vi "Search.vi"() -> (8 "data":string[][](array[string]), 10 "Leds":bool[](array[boolean]))   [LabVIEW 2021]
uses:
  <vilib>/addons/_office/excel.llb/Excel Get Data ([str]).vi
  <vilib>/Utility/NIReport.llb/NI_report.lvclass
  <vilib>/Utility/NIReport.llb/Excel/NI_Excel.lvclass
  <vilib>/addons/_office/NI_ReportGenerationToolkit.lvlib
panel:
  in  "Check":bool
  in  "Saisir des chiffres\nvérifier":string[](array[string])
  out "data string":string[][](array[string])
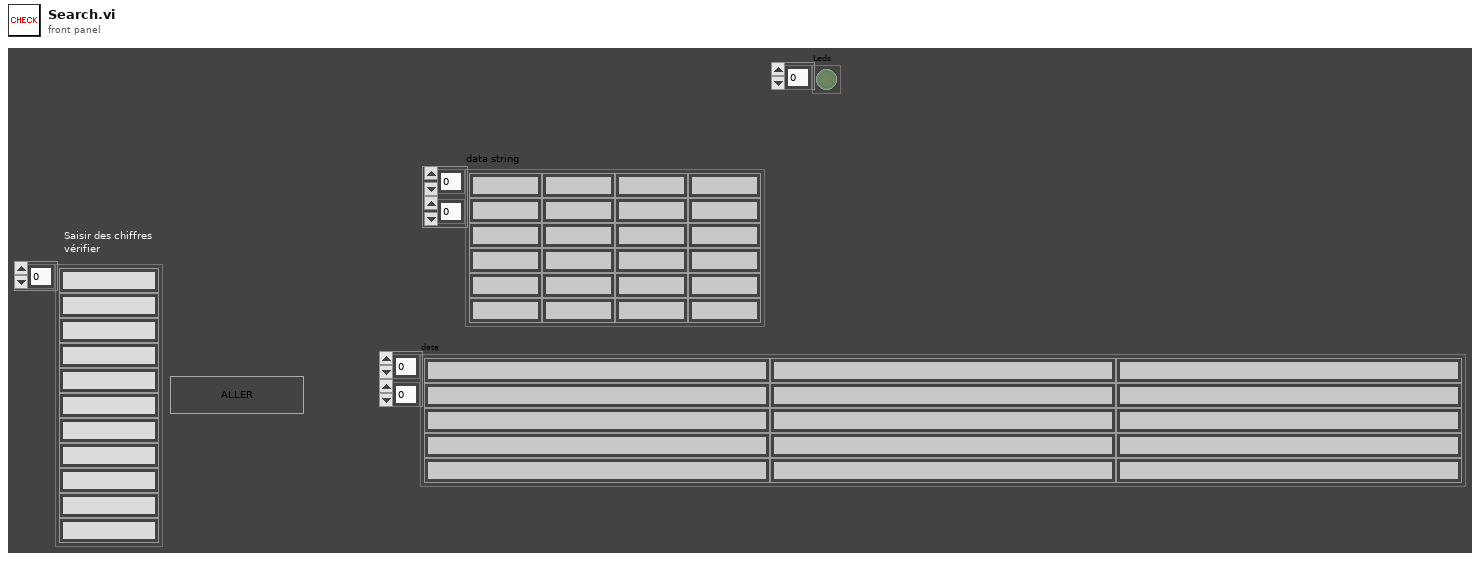
[diagram p1: front panel]
types:
  T1 = enum16{"Standard Report", "HTML", "Word", "Excel"}
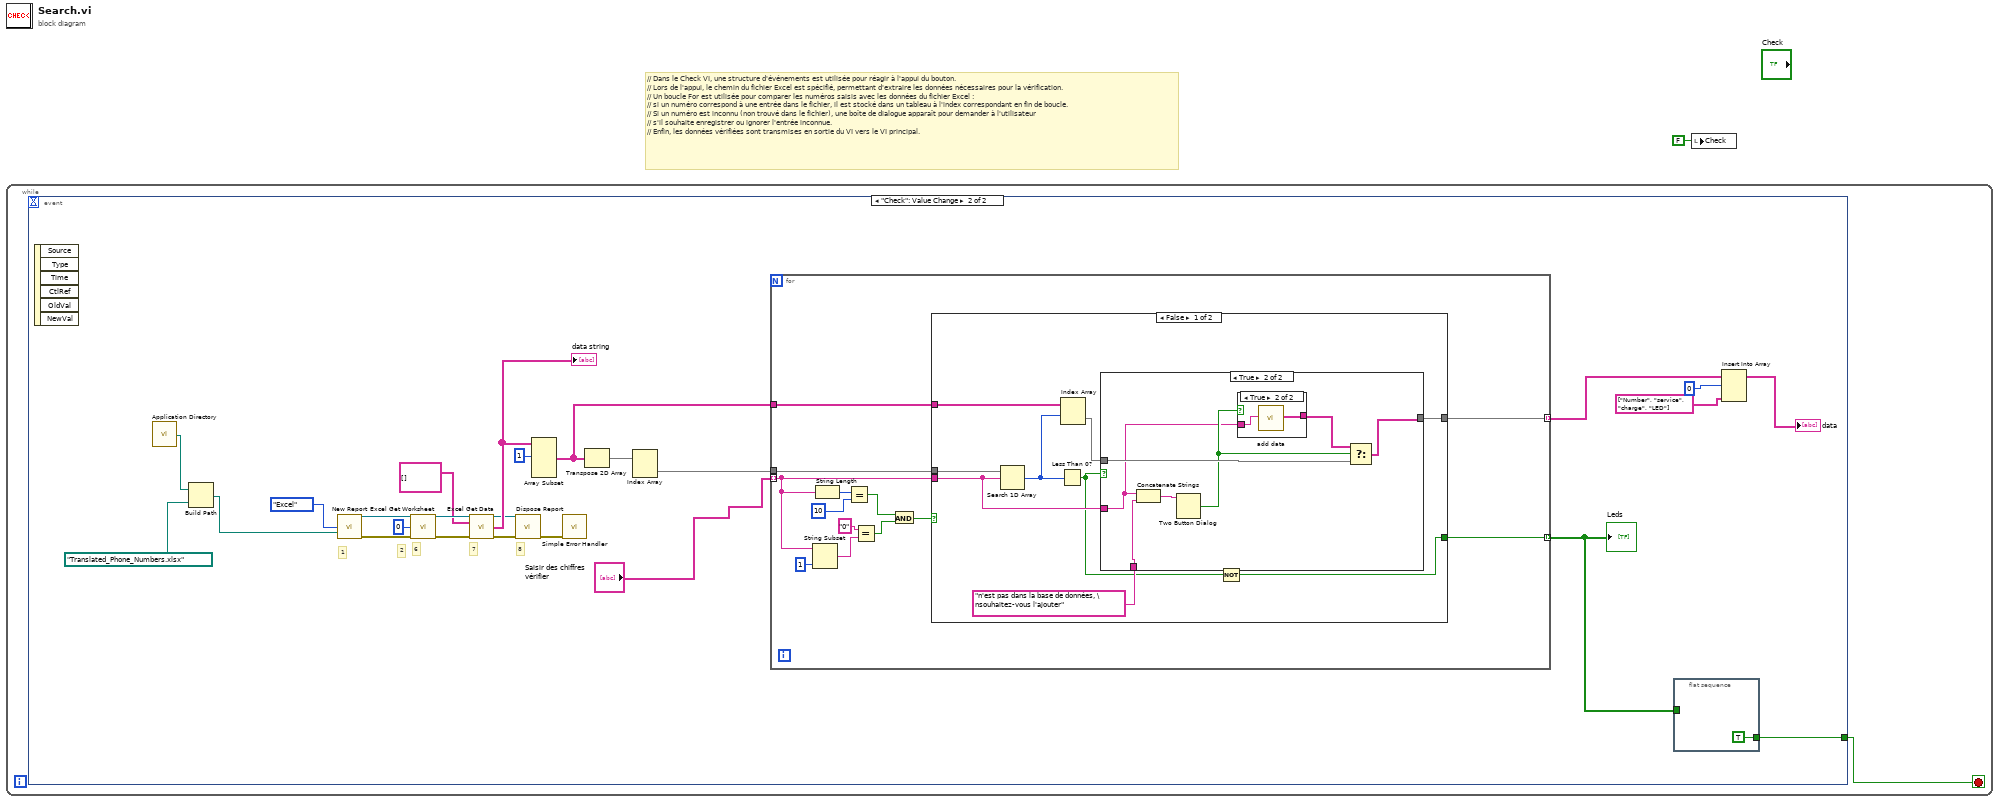
[diagram p0: block diagram]
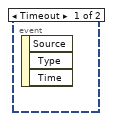
[diagram p2: hidden frame]
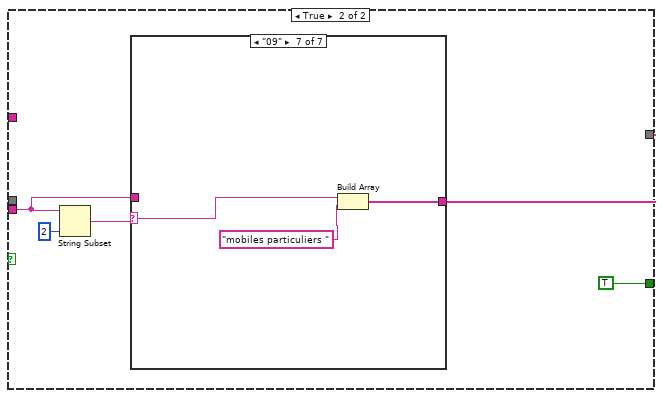
[diagram p5: hidden frame]
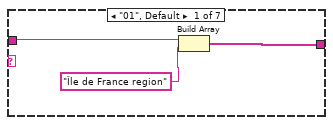
[diagram p6: hidden frame]
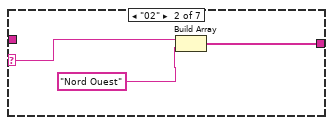
[diagram p7: hidden frame]
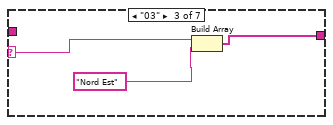
[diagram p8: hidden frame]
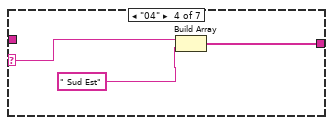
[diagram p9: hidden frame]
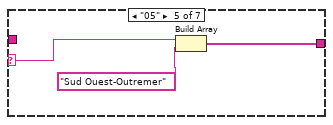
[diagram p10: hidden frame]
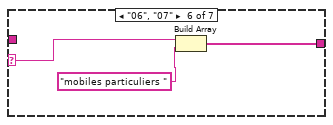
[diagram p11: hidden frame]
diagram:
  # "// Dans le Check VI, une structure d'événements est utilisée pour réagir à l'appui du bouton.\n// Lors de l'appui, le chemin du fichier Excel est spécifié, permettant d'extraire les données nécessaires pour la vérification.\n// Un boucle For est utilisée pour comparer les numéros saisis avec les données du fichier Excel : \n// si un numéro correspond à une entrée dans le fichier, il est stocké dans un tableau à l'index correspondant en fin de boucle.\n// Si un numéro est inconnu (non trouvé dans le fichier), une boîte de dialogue apparaît pour demander à l'utilisateur \n// s'il souhaite enregistrer ou ignorer l'entrée inconnue.\n// Enfin, les données vérifiées sont transmises en sortie du VI vers le VI principal."
  n1 = while {
    stop <- w2 stop-if-true
    n2 = event shown="[1] \"Check\": Value Change" {
      selector: _ -> [_ _]
      dyn-events: _ -> [_ _]
      timeout: _ -> [_ _]
      tunnel: [_ w7] -> w2
      event Timeout {
        n3 = event-data() -> ()  [unwired: 1 in, 3 out]
      }
      event "Check": Value Change {
        # "8"
        # "7"
        # "6"
        # "2"
        # "1"
        n4 = event-data() -> ()  [unwired: 1 in, 6 out]
        n5 = call <vilib>:"Application Directory.vi"() -> ("Application Directory"=w5:path)
        n6 = Build Path(base path=w5, name or relative path=path "Translated_Phone_Numbers.xlsx") -> (appended path=w3:path)
        n7 = call <vilib>:"New Report.vi"("report type"=T1."Excel", "template (empty)"=w3) -> ("report out"=w19:refnum<class "NI_report.lvclass">, "error out"=w20:errorcluster)  [unwired: 12 in]
        n8 = call <vilib>:"Excel Get Worksheet.vi"("report in"=w19, "worksheet index (0)"=0, "error in (no error)"=w20) -> ("report out"=w15:refnum<class "NI_report.lvclass">, "error out"=w14:errorcluster)  [unwired: 11 in]
        n9 = call-poly <vilib>:"Excel Get Data.vi"("report in"=w15, "data type"=string[][] [], "error in (no error)"=w14) -> ("report out"=w16:refnum<class "NI_report.lvclass">, "data"=w23:string[][], "error out"=w17:errorcluster)  [unwired: 10 in]
        "data string" <- w23
        n10 = call-dynamic "Dispose Report.vi"("report in"=w16, "error in (no error)"=w17) -> ("error out"=w18:errorcluster)  [unwired: 13 in]
        n11 = Array Subset(array=w23, index (row)=1 ("index")) -> (w24:string[][])  [unwired: 3 in]
        n12 = call <vilib>:"Simple Error Handler.vi"("error in (no error)"=w18) -> ()  [unwired: 4 in, 5 out]
        n13 = Transpose 2D Array(2D array=w24) -> (transposed array=w21:string[][])
        n14 = Index Array(array=w21) -> (element=w22:string[])  [unwired: 2 in]
        n15 = for {
          tunnel: w22 -> [w41]
          tunnel: "Saisir des chiffres\nvérifier" -> [w34] mode=indexing
          tunnel: w24 -> [w40]
          tunnel: [w39] -> w25 mode=indexing
          tunnel: [w29] -> w6 mode=indexing
          n16 = String Subset(string=w34, length (rest)=1 ("length (rest)")) -> (substring=w37:string)  [unwired: 1 in]
          n17 = String Length(string=w34) -> (length=w33:i32)
          n18 = Equal?(x=w33, y=10) -> (x = y?=w31:bool)
          n19 = Equal?(x="0", y=w37) -> (x = y?=w35:bool)
          n20 = And(x=w31, y=w35) -> (x .and. y?=w30:bool)
          n21 = case shown="False" w30 {
            tunnel: w41 -> [w50 _]
            tunnel: w34 -> [w47 w62]
            tunnel: w40 -> [w49 _]
            tunnel: [w44 w63] -> w39
            tunnel: [w42 TRUE] -> w29
            frame False {
              n22 = Search 1D Array(1D array=w50, element=w47) -> (index of element=w48:i32)  [unwired: 1 in]
              n23 = Less Than 0?(x=w48) -> (x < 0?=w43:bool)
              n24 = Index Array(array=w49, index (row)=w48) -> (element=w45:string[])  [unwired: 1 in]
              n25 = case shown="True" w43 {
                tunnel: w47 -> [_ w52]
                tunnel: "n'est pas dans la base de données, \nsouhaitez-vous l'ajouter" ("string") -> [_ w58]
                tunnel: w45 -> [w51 w56]
                tunnel: [w51 w55] -> w44
                frame False {
                }
                frame True {
                  n26 = Concatenate Strings(w52, w58) -> (w57:string)
                  n27 = Two Button Dialog(message=w57) -> (T button?=w53:bool)  [unwired: 2 in]
                  n28 = case shown="True" w53 {
                    tunnel: [_ w60] -> w54
                    tunnel: w52 -> [_ w59]
                    frame False {
                    }
                    frame True {
                      n29 = call "add data.vi"("nombre"=w59) -> ("New Data"=w60:string[])  [unwired: 10 in]
                    }
                  }
                  n30 = Select(t=w54, s=w53, f=w56) -> (s? t:f=w55:string[])
                }
              }
              n31 = Not(x=w43) -> (.not. x?=w42:bool)
            }
            frame True {
              n32 = String Subset(string=w62, length (rest)=2 ("length (rest)")) -> (substring=w64:string)  [unwired: 1 in]
              n33 = case shown="\"09\"" w64 {
                selector: w64 -> [_ w71 w74 w77 w80 w83 w86]
                tunnel: [w67 w69 w72 w75 w78 w81 w84] -> w63
                tunnel: w62 -> [w66 _ _ _ _ _ _]
                frame "01", Default {
                  n34 = Build Array(w66, "Île de France region") -> (w67:string[])
                }
                frame "02" {
                  n35 = Build Array(w71, "Nord Ouest") -> (w69:string[])
                }
                frame "03" {
                  n36 = Build Array(w74, "Nord Est") -> (w72:string[])
                }
                frame "04" {
                  n37 = Build Array(w77, " Sud Est") -> (w75:string[])
                }
                frame "05" {
                  n38 = Build Array(w80, "Sud Ouest-Outremer") -> (w78:string[])
                }
                frame "06", "07" {
                  n39 = Build Array(w83, "mobiles particuliers ") -> (w81:string[])
                }
                frame "09" {
                  n40 = Build Array(w86, "mobiles particuliers ") -> (w84:string[])
                }
              }
            }
          }
        }
        "Leds" <- w6
        n41 = flat-sequence {
          tunnel: [TRUE] -> w7
          tunnel: w6 -> [_]
          frame #0 {
          }
        }
        n42 = Insert Into Array(array=w25, index (row)=0, new element=string[] ["Number", "service", "charge", "LED"] ("new element/subarray")) -> (→"data":string[][])  [unwired: 1 in]
      }
    }
  }
  n43 = local write "Check"(FALSE ("Check")) -> ()
